vi "IMES.vi"(2 "Boolean":bool=TRUE, 5 "error in (no error)":errorcluster, 6 "Measured voltage":string, 8 "Measured":string, 10 "HI SET":string, 12 "LO SET":string) -> (19 "error out":errorcluster)   [LabVIEW 2021]
uses:
  Template/Main_VI/Control/Ini.ctl
  <vilib>/httpClient/LabVIEWHTTPClient.lvlib
panel:
  out "concatenated string 2":string
  out "concatenated string":string
  out "standard output":string
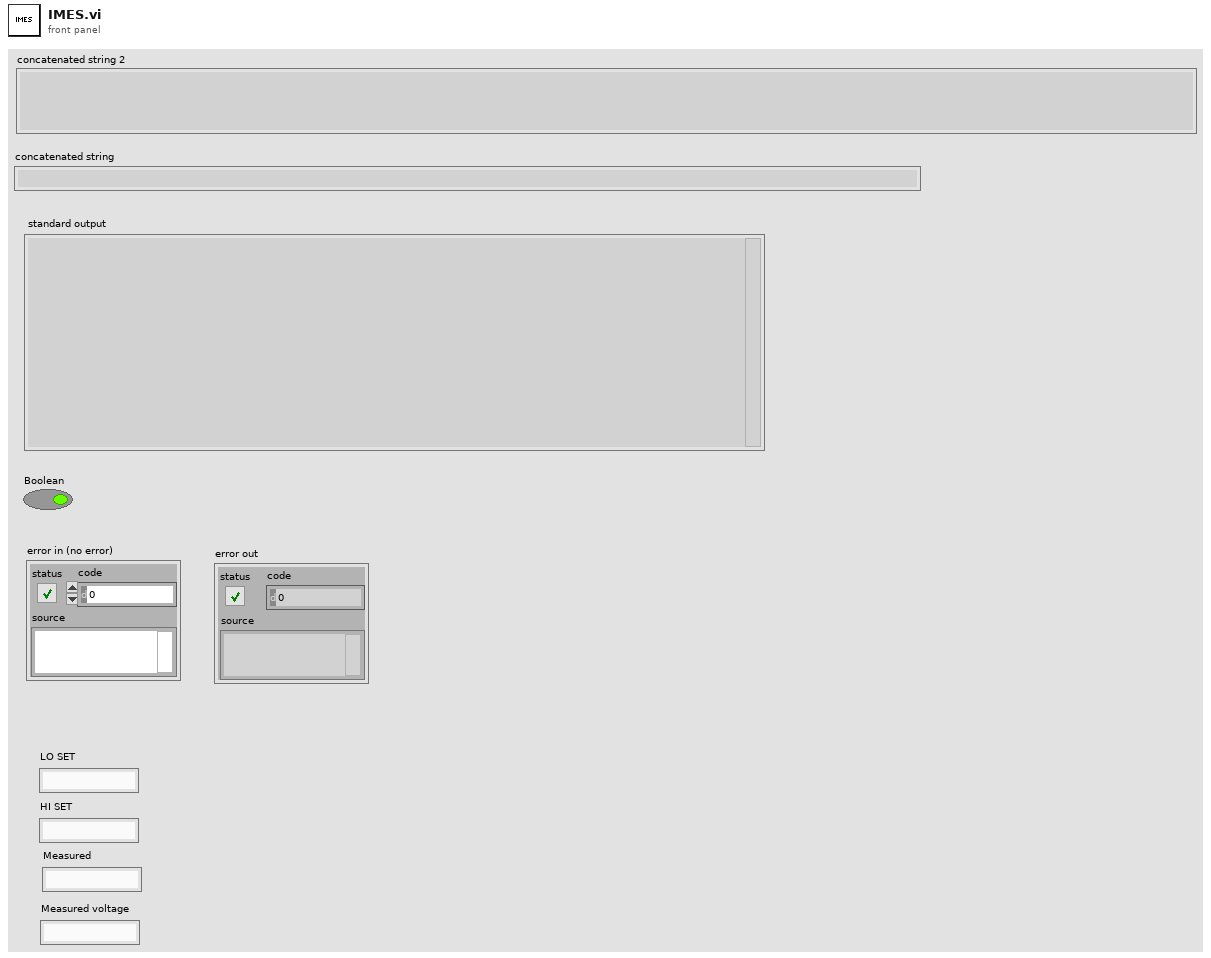
[diagram p1: front panel]
types:
  T1 = typedef "Ini.ctl" = enum16{"Write", "Read"}
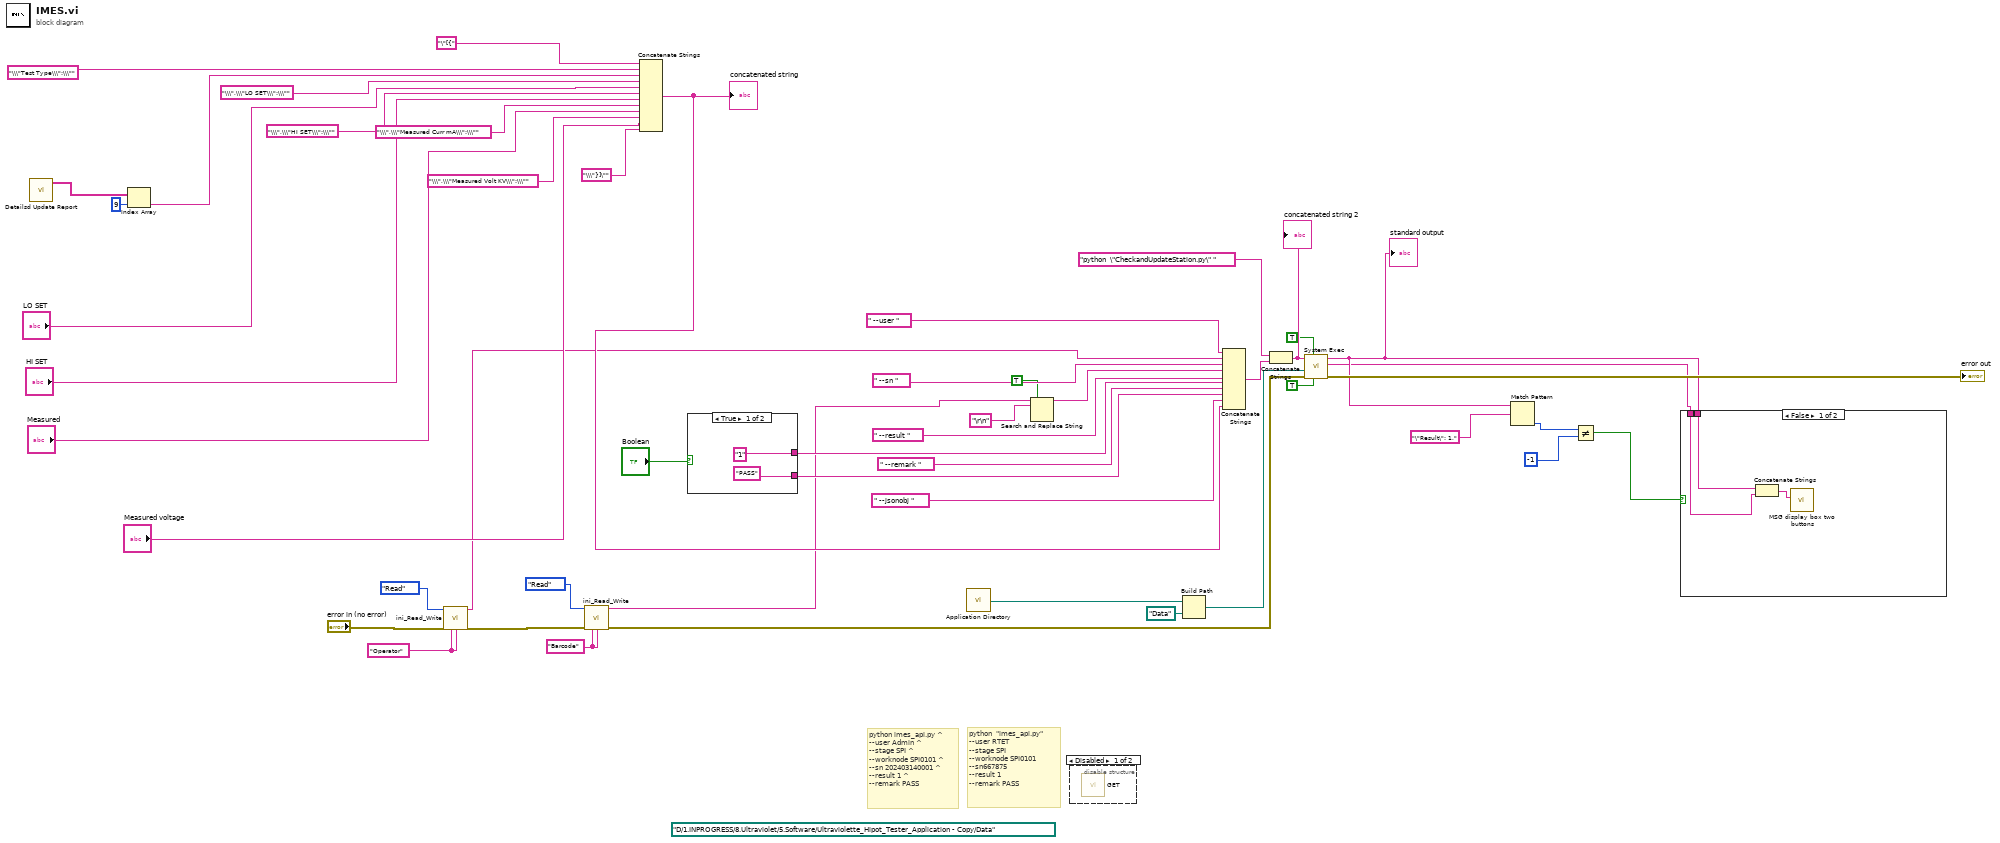
[diagram p0: block diagram]
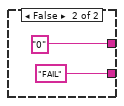
[diagram p4: hidden frame]
diagram:
  w39 = "Operator" ("Write Section")
  w40 = "Barcode" ("Write Section")
  (unwired) path "D:/1.INPROGRESS/8.Ultraviolet/5.Software/Ultraviolette_Hipot_Tester_Application - Copy/Data" ("working directory")
  # "python  \"imes_api.py\" \n--user RTET \n--stage SPI \n--worknode SPI0101 \n--sn667875 \n--result 1 \n--remark PASS"
  # "python imes_api.py ^\n--user Admin ^\n--stage SPI ^\n--worknode SPI0101 ^\n--sn 202403140001 ^\n--result 1 ^\n--remark PASS"
  n1 = call "Detailsd Update Report.vi"() -> ("appended array"=w22:string[])  [unwired: 11 in]
  n2 = Index Array(array=w22, index=9) -> (element=w18:string)
  n3 = call "ini_Read_Write.vi"(0:Ini."Read", "error in (no error) 2"="error in (no error)", "Read Section"=w39, "Read Key"=w39) -> ("value"=w2:string, "error in (no error) 3"=w37:errorcluster)  [unwired: 10 in]
  n4 = call "ini_Read_Write.vi"(0:Ini."Read", "error in (no error) 2"=w37, "Read Section"=w40, "Read Key"=w40) -> ("value"=w1:string, "error in (no error) 3"=w35:errorcluster)  [unwired: 10 in]
  n5 = Concatenate Strings("\"[{" ("string"), "\\\"Test Type\\\":\\\"" ("string"), w18, "\\\",\\\"LO SET\\\":\\\"" ("string"), "LO SET", "\\\",\\\"HI SET\\\":\\\"" ("string"), "HI SET", "\\\",\\\"Measured Curr mA\\\":\\\"" ("string"), "Measured", "\\\",\\\"Measured Volt KV\\\":\\\"" ("string"), "Measured voltage", "\\\"}]\"" ("string")) -> (w3:string)
  "concatenated string" <- w3
  n6 = case shown="True" "Boolean" {
    tunnel: ["PASS" ("string") "FAIL" ("string")] -> w23
    tunnel: ["1" ("string") "0" ("string")] -> w25
    frame True {
    }
    frame False {
    }
  }
  n7 = call <vilib>:"Application Directory.vi"() -> ("Application Directory"=w44:path)
  n8 = Search and Replace String(replace all?=TRUE ("replace all? (F)"), input string=w1, search string="\r\n") -> (result string=w5:string)  [unwired: 5 in, 3 out]
  n9 = disable-structure shown="Disabled" {
    frame Disabled {
      n10 = call <vilib>:"GET.vi"() -> ()  [unwired: 12 in, 4 out]
    }
    frame Enabled {
    }
  }
  n11 = Build Path(base path=w44, name or relative path=path "Data") -> (appended path=w43:path)
  n12 = Concatenate Strings(" --user " ("string"), w2, " --sn " ("string"), w5, " --result " ("string"), w25, " --remark " ("string"), w23, " --jsonobj " ("string"), w3) -> (w48:string)
  n13 = Concatenate Strings("python  \"CheckandUpdateStation.py\" " ("command line"), w48) -> (w49:string)
  "concatenated string 2" <- w49
  n14 = call <vilib>:"System Exec.vi"("run minimized? (F)"=TRUE, "wait until completion? (T)"=TRUE, "error in (no error)"=w35, "working directory"=w43, "command line"=w49) -> ("error out"=→"error out":errorcluster, "standard error"=w8:string, "standard output"=w26:string)  [unwired: 3 in, 1 out]
  "standard output" <- w26
  n15 = Match Pattern(string=w26, regular expression="\"Result\": 1,") -> (offset past match=w30:i32)  [unwired: 1 in, 3 out]
  n16 = Not Equal?(x=w30, y=-1) -> (x != y?=w27:bool)
  n17 = case shown="False" w27 {
    tunnel: w26 -> [w57 _]
    tunnel: w8 -> [w56 _]
    frame False {
      n18 = Concatenate Strings(w57, w56) -> (w55:string)
      n19 = call "MSG display box two buttons.vi"("input string"=w55) -> ()  [unwired: 8 in, 3 out]
    }
    frame True {
    }
  }
